vi "GetWindowLongPtrW Wrapper Template.vi"(0 "hWnd":u64, 5 "nIndex":i32=-16, 11 "error in":errorcluster) -> (4 "return value":i64, 15 "error out":errorcluster)   [LabVIEW 2020]
doc: "Reads a value of the window hWnd through user32.dll GetWindowLongPtrW (stdcall, called in any thread). nIndex -16 GWL_STYLE returns the window style (WS_POPUP 0x80000000, WS_CAPTION 0x00C00000, WS_VISIBLE 0x10000000); -20 GWL_EXSTYLE the extended style. 0 can mean failure. When error in carries an error the DLL is not called. Generated by scripts\\Build Win32 Wrappers.vi - do not edit by hand, rebuild it."
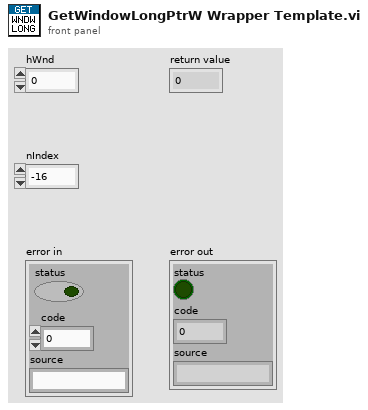
[diagram p1: front panel]
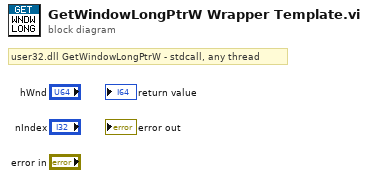
[diagram p0: block diagram]
diagram:
  # "user32.dll GetWindowLongPtrW - stdcall, any thread"
